vi "UpdateToolbar.vi"(1 "ToolbarButtons":T1[](array[typedef]), 5 "error in (no error)":errorcluster) -> (19 "error out":errorcluster)   [LabVIEW 2020, in "UmlEditor.lvclass"]
uses:
  <resource>/Framework/Providers/Open_GDS/UML/UmlEditor_class/UmlEditor.lvclass
  <resource>/Framework/Providers/Open_GDS/UML/Graph_class/ToolbarButtonType.ctl
  <resource>/Framework/Providers/Open_GDS/UML/UMLEditor/UMLEditor tooltype.ctl
  <resource>/Framework/Providers/Open_GDS/UML/Graph_class/Graph.lvclass
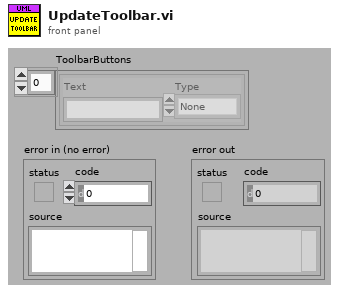
[diagram p1: front panel]
types:
  T1 = typedef "Graph.lvclass/ToolbarButtonType.ctl" = cluster{"Text":string, "Type":T2}
  T2 = typedef "UMLEditor tooltype.ctl" = enum16{"None", "Node", "Edge"}
  T3 = typedef "UmlEditor.lvclass/ObjectAttributes.ctl" = cluster{"ListeningQueueIn":refnum<queue>, "Event":refnum<user-event>, "UseProjectFolderAsBasePath":bool, "TypeSyncOption":bool, "Attr":string[], "ToolTip":cluster{"ToolTipOpen":bool, "LastToolTip":i32}, "ClassesToIgnore":string[], "UndoSize":i32, "OpenLastSavedFileWhenStarting":bool, "SyncOption":T4, "SyncTime(s)":i32, "Params":cluster{"IniParams":T5, "Value":string}[], "GraphButtons":refnum<vi>}
  T4 = typedef "UMLEditor_SyncOptions.ctl" = cluster{"IgnoreInstrLib":bool, "IgnoreUserLib":bool, "IgnoreViLib":bool}
  T5 = typedef "UmlEditor.lvclass/IniParamsType.ctl" = enum16{"I have problem with UML stability on my computer"}
  T6 = cluster{"left":i16, "top":i16, "right":i16, "bottom":i16}
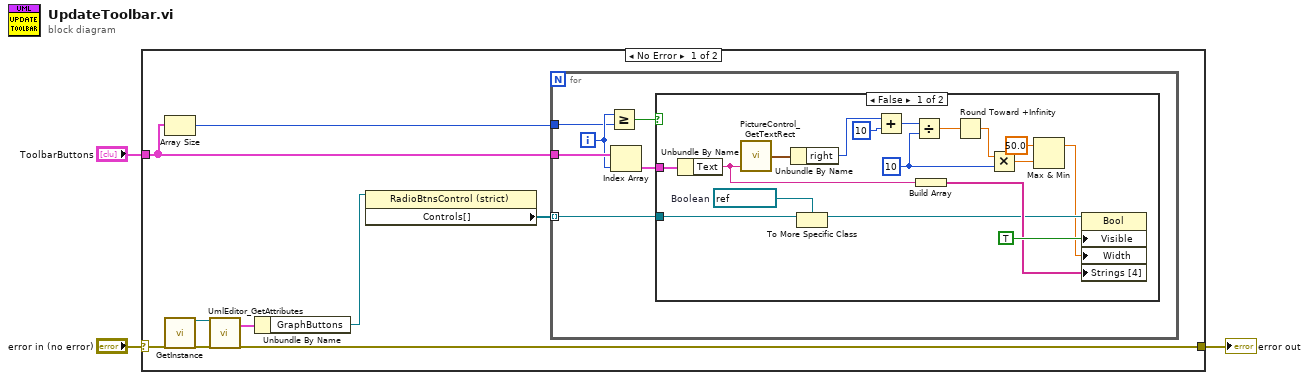
[diagram p0: block diagram]
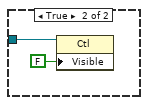
[diagram p2: hidden frame]
diagram:
  n1 = case shown="No Error" "error in (no error)" {
    selector: "error in (no error)" -> [w8 w38]
    tunnel: [w11 w38] -> w2
    tunnel: "ToolbarButtons" -> [w5 _]
    frame No Error {
      n2 = Array Size(array=w5) -> (size(s)=w4:i32)
      n3 = call <resource>:"GetInstance.vi"("error in (no error)"=w8) -> ("reference out"=w10:refnum<class "UmlEditor.lvclass">, "error out"=w9:errorcluster)  [unwired: 17 out]
      n4 = call <resource>:"UmlEditor_GetAttributes.vi"("reference in"=w10, "error in (no error)"=w9) -> ("Data"=w12:T3, "error out"=w11:errorcluster)  [unwired: 14 in, 2 out]
      n5 = Unbundle By Name(w12) -> ("GraphButtons"=w7:refnum<vi>)
      n6 = property class="RadioBtnsControl (strict)"(reference=w7) -> ("Controls[]"=w6:refnum<vi>[])  [unwired: 1 in, 2 out]
      n7 = for {
        tunnel: w6 -> [w14] mode=indexing
        tunnel: w5 -> [w18]
        tunnel: w4 -> [w16]
        i -> [w17]
        n8 = Greater Or Equal?(x=w17, y=w16) -> (x >= y?=w15:bool)
        n9 = Index Array(array=w18, index=w17) -> (element=w13:T1)
        n10 = case shown="False" w15 {
          tunnel: w14 -> [w23 w37]
          tunnel: w13 -> [w33 _]
          frame False {
            w24 = refnum<vi> refnum  # Boolean
            w26 = i16 10 ("y")
            n11 = Unbundle By Name(w33) -> ("Text"=w31:string)
            n12 = call <resource>:"PictureControl_GetTextRect.vi"("text"=w31) -> ("rect"=w32:T6)  [unwired: 8 in]
            n13 = Unbundle By Name(w32) -> ("right"=w30:i16)
            n14 = To More Specific Class(target class=w24, reference=w23) -> (specific class reference=w22:refnum<vi>)  [unwired: 1 in, 1 out]
            n15 = Add(x=w30, y=i16 10) -> (x+y=w28:i16)
            n16 = Divide(x=w28, y=w26) -> (x/y=w27:dbl)
            n17 = Build Array(w31) -> (w34:string[])
            n18 = Round Toward +Infinity(x=w27) -> (ceil(x): smallest int >= x=w25:dbl)
            n19 = Multiply(x=w25, y=w26) -> (x*y=w21:dbl)
            n20 = Max & Min(x=50.0, y=w21) -> (max(x,y)=w20:dbl)  [unwired: 1 out]
            n21 = property class="Bool"(reference=w22, "Visible"=TRUE, "Width"=w20, "Strings [4]"=w34) -> ()  [unwired: 1 in, 2 out]
          }
          frame True {
            n22 = property class="Ctl"(reference=w37, "Visible"=FALSE) -> ()  [unwired: 1 in, 2 out]
          }
        }
      }
    }
    frame Error {
    }
  }
  "error out" <- w2
